vi "_Raise Dom Content Loaded.vi"(4 "WebView2.lvlib:WebView2 Control.lvclass":refnum<class "WebView2 Control.lvclass">, 5 "Event Data":cluster{"sender":refnum<k24>, "e":refnum<k24>}, 6 "Control Ref":refnum<k24>, 7 "Event Common Data":T1) -> ()   [LabVIEW 2020, in "WebView2.lvlib" / "WebView2 Control.lvclass"]
uses:
  WebView2 Control.lvclass
  E:/Labview/LV 2023/PPL/PPL Builder/Libs/LV-WebView2/Source/Libs/Microsoft.Web.WebView2.Core.dll
  Libs/Microsoft.Web.WebView2.Core.dll
  WebView2 Control.lvclass/WebView2 Control.ctl
  WebView2 Event Filter Interface/WebView2 Event Filter Interface.lvclass
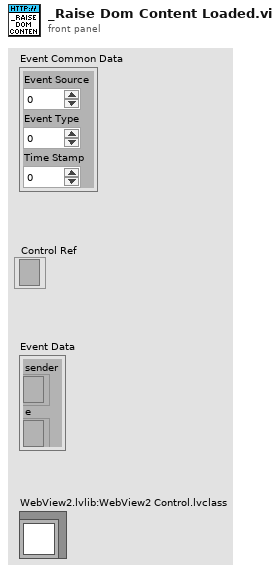
[diagram p1: front panel]
types:
  T1 = cluster{"Event Source":i32, "Event Type":u32, "Time Stamp":u32}
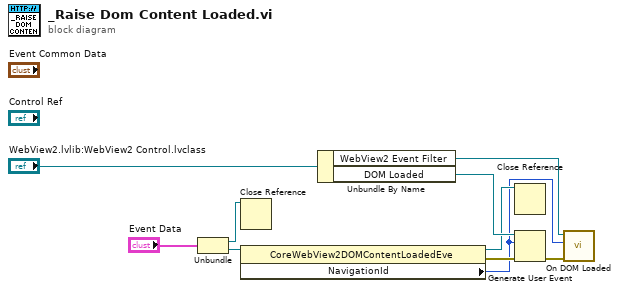
[diagram p0: block diagram]
diagram:
  n1 = Unbundle("Event Data") -> ("sender"=w5:refnum<k24>, "e"=w7:refnum<k24>)
  n2 = Close Reference(reference=w5) -> ()  [unwired: 1 in, 1 out]
  n3 = property class="CoreWebView2DOMContentLoadedEve"(reference=w7) -> (reference out=w4:refnum<k24>, error out=w6:errorcluster, "NavigationId"=w2:u64)  [unwired: 1 in]
  n4 = Unbundle By Name("WebView2.lvlib:WebView2 Control.lvclass") -> ("WebView2 Event Filter"=w3:refnum<class "WebView2 Event Filter Interface.lvclass">, "DOM Loaded"=w9:refnum<user-event>)
  n5 = Close Reference(reference=w4) -> ()  [unwired: 1 in, 1 out]
  n6 = Generate User Event(user event=w9, event data cluster=w2, error in=w6) -> (error out=w1:errorcluster)  [unwired: 1 in, 1 out]
  n7 = call-dynamic "On DOM Loaded.vi"("error in (no error)"=w1, "NavigationId"=w2, "WebView2 Event Filter Interface in"=w3) -> ()  [unwired: 8 in, 1 out]
